vi "FuncVI-Decimate.vi"(5 "InstanceRef":T2, 9 "arg list":T1[](array[typedef]) {"num" format="%.2f"}) -> (0 "error out":bool, 3 "result":T1 {"num" format="%.2f"})   [LabVIEW 2021]
doc: "::: CalcExpress Toolkit :::\nCopyright (c) 2000-2026 Konstantin Shifershteyn. All rights reserved."
uses:
  cetypes.llb/CalcExpress Function Argument Info.ctl
  cetypes.llb/CalcExpress Instance RefNum.ctl
  <vilib>/Analysis/2dsp.llb/Decimate (single shot, DBL).vi
  <vilib>/Analysis/NI_AALPro.lvlib
panel:
  in  "max arg num":i32=3
  in  "min arg num":i32=1
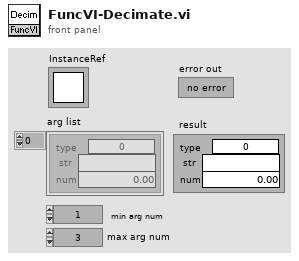
[diagram p1: front panel]
types:
  T1 = typedef "CalcExpress Function Argument Info.ctl" = cluster{"type":u32, "str":string, "num":dbl}
  T2 = typedef "CalcExpress Instance RefNum.ctl" = refnum<k1>
  T3 = enum8{"String", "DBL Number", "identifier", "1D Array of DBL", "2D Array of DBL", "CDB Number", "1D Array of CDB", "2D Array of CDB", "1D Array of String", "2D Array of String", "Unknown data type"}
  T4 = cluster{"index":i32, "type":enum8{"String", "DBL Number", "identifier", "1D Array of DBL", "2D Array of DBL", "CDB Number", "1D Array of CDB", "2D Array of CDB", "Unknown data type"}, "default num":dbl, "default str":string}[]
  T5 = cluster{"type":enum8{"String", "DBL Number", "identifier", "1D Array of DBL", "2D Array of DBL", "CDB Number", "1D Array of CDB", "2D Array of CDB", "1D Array of String", "2D Array of String", "Unknown data type"}, "data string":string, dbl}
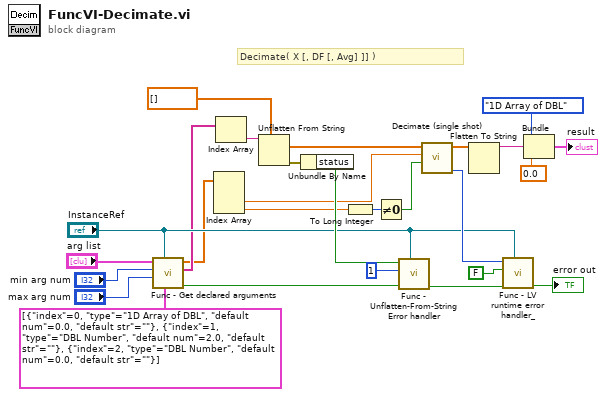
[diagram p0: block diagram]
diagram:
  # "Decimate( X [, DF [, Avg] ]] )"
  n1 = call "Func - Get declared arguments.vi"("arg descriptors"=T4 [{"index"=0, "type"=enum."1D Array of DBL", "default num"=0.0, "default str"=""}, {"index"=1, "type"=enum."DBL Number", "default num"=2.0, "default str"=""}, {"index"=2, "type"=enum."DBL Number", "default num"=0.0, "default str"=""}] ("args descriptors"), "InstanceRef"="InstanceRef", "max arg num"="max arg num", "min arg num"="min arg num", "arg list"="arg list") -> ("error out"=w14:bool, "str list"=w4:string[], "num list"=w3:dbl[])  [unwired: 3 in, 1 out]
  n2 = Index Array(array=w3) -> (element #2=w2:dbl, element #3=w1:dbl)  [unwired: 3 in, 1 out]
  n3 = Index Array(array=w4) -> (element=w17:string)  [unwired: 1 in]
  n4 = Unflatten From String(type=dbl[] [] ("num list"), binary string=w17) -> (value=w18:dbl[], error out=w6:errorcluster)  [unwired: 3 in, 1 out]
  n5 = Unbundle By Name(w6) -> ("status"=w13:bool)
  n6 = To Long Integer(number=w1) -> (32bit integer=w9:i32)
  n7 = Not Equal To 0?(x=w9) -> (x != 0?=w16:bool)
  n8 = call "Func - Unflatten-From-String Error handler.vi"("InstanceRef"="InstanceRef", "error in"=w14, "argument number"=1, "Unflatten Error status"=w13) -> ("error out"=w10:bool)  [unwired: 5 in]
  n9 = call-poly <vilib>:"Decimate (single shot).vi"("averaging"=w16, "decimating factor"=w2, "X"=w18) -> ("error"=w22:i32, "Decimated Array"=w21:dbl[])  [unwired: 7 in]
  n10 = Flatten To String(anything=w21) -> (data string=w20:string)  [unwired: 3 in, 2 out]
  n11 = call "Func - LV runtime error handler_.vi"("InstanceRef"="InstanceRef", "error in"=w10, "Gen CE error?"=FALSE, "LabVIEW error code"=w22) -> ("error out"=→"error out":bool)  [unwired: 7 in]
  n12 = Bundle("type"=T3."1D Array of DBL", "data string"=w20, 0.0) -> (→"result":T5)  [unwired: 1 in]
